vi "Read View VI and FP Refs.vi"(0 "GUI Container in":refnum<class "GUI Container.lvclass">, 5 "View":string, 7 "View Hierarchy Level":i32, 11 "error in (no error)":errorcluster) -> (4 "GUI Container out":refnum<class "GUI Container.lvclass">, 6 "View Status":T1, 8 "VI References":T4, 10 "View Found":bool, 15 "error out":errorcluster)   [LabVIEW 2023, in "GUI Views.lvlib" / "GUI Container.lvclass"]
uses:
  GUI Container.lvclass
  typedefs/VI References.ctl
  typedefs/View Status.ctl
  <vilib>/ActorFramework/Message Enqueuer/Message Enqueuer.lvclass
  typedefs/View Details.ctl
  typedefs/FP Status.ctl
  GUI Container.lvclass/GUI Container.ctl
  <vilib>/ErrorRing/Error Ring.xnode
  <vilib>/Utility/error.llb/Error Cluster From Error Code.vi
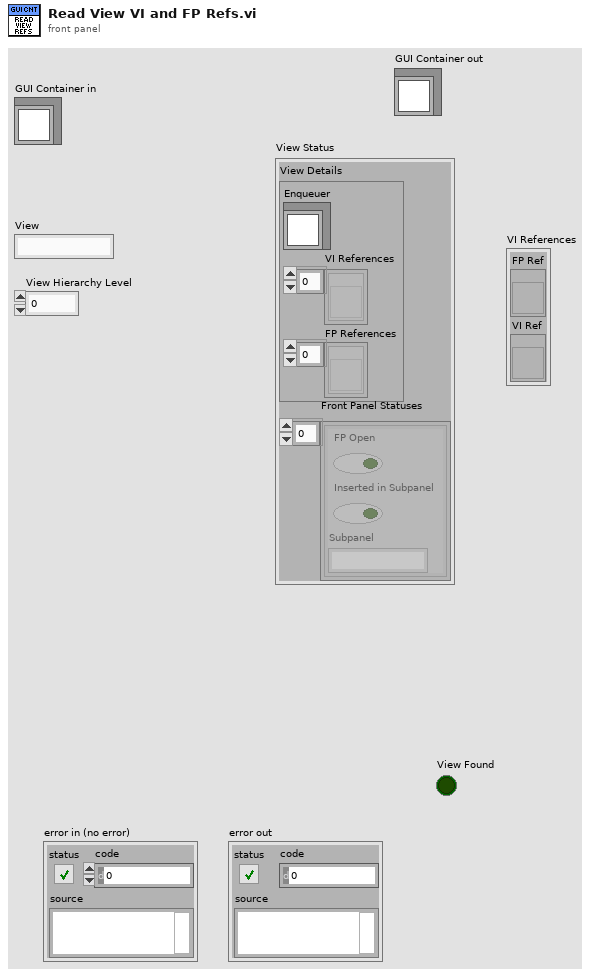
[diagram p1: front panel]
types:
  T1 = typedef "GUI Views.lvlib/GUI Container.lvclass/View Status.ctl" = cluster{"View Details":T2, "Front Panel Statuses":T3[]}
  T2 = typedef "GUI Views.lvlib/GUI Container.lvclass/View Details.ctl" = cluster{"Enqueuer":refnum<class "Message Enqueuer.lvclass">, "VI References":refnum<vi>[], "FP References":refnum<vi>[]}
  T3 = typedef "GUI Views.lvlib/GUI Container.lvclass/FP Status.ctl" = cluster{"FP Open":bool, "Inserted in Subpanel":bool, "Subpanel":string}
  T4 = typedef "GUI Views.lvlib/GUI Container.lvclass/VI References.ctl" = cluster{"FP Ref":refnum<vi>, "VI Ref":refnum<vi>}
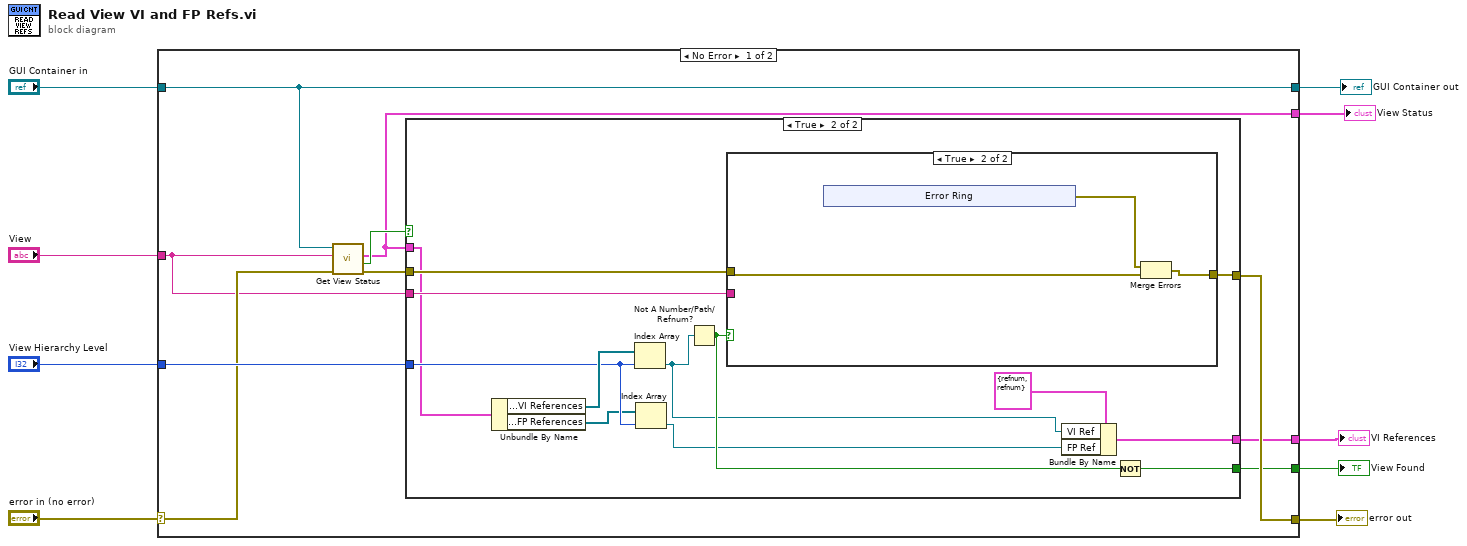
[diagram p0: block diagram]
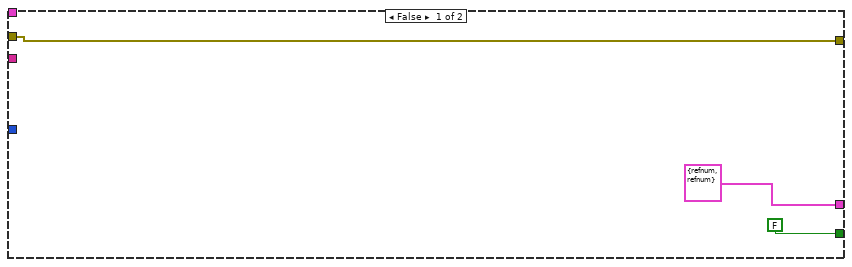
[diagram p2: hidden frame]
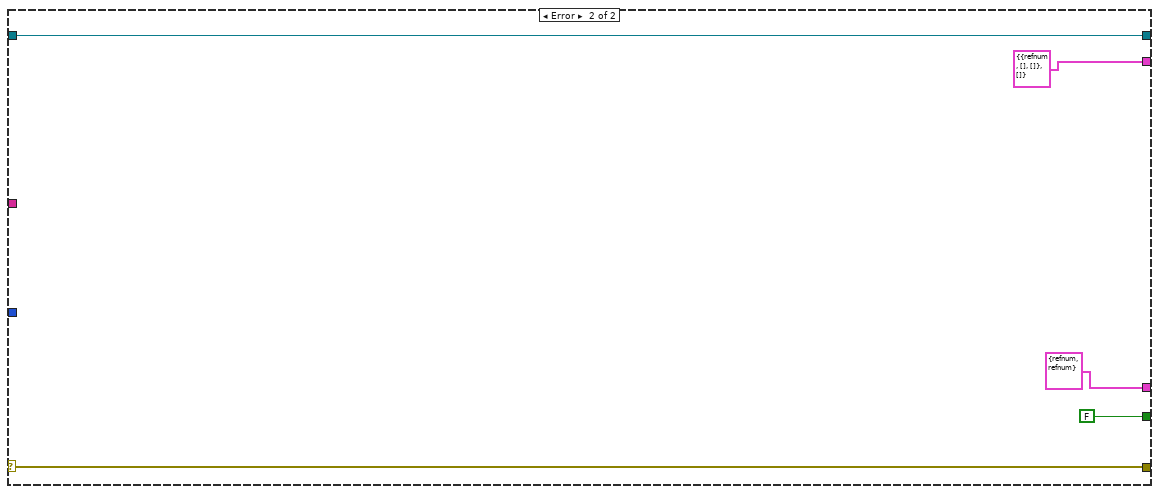
[diagram p4: hidden frame]
diagram:
  n1 = case shown="No Error" "error in (no error)" {
    selector: "error in (no error)" -> [w16 w47]
    tunnel: [w19 w47] -> w9
    tunnel: "GUI Container in" -> [w13 w48]
    tunnel: "View Hierarchy Level" -> [w18 _]
    tunnel: "View" -> [w14 _]
    tunnel: [w13 w48] -> w4
    tunnel: [w17 FALSE] -> w3
    tunnel: [w11 T4 {"FP Ref"=refnum, "VI Ref"=refnum} ("VI References")] -> w2
    tunnel: [w10 T1 {"View Details"={"Enqueuer"=refnum, "VI References"=[], "FP References"=[]}, "Front Panel Statuses"=[]} ("View State")] -> w1
    frame No Error {
      n2 = call "Get View Status.vi"("error in (no error)"=w16, "View"=w14, "GUI Container View in"=w13) -> ("error out"=w15:errorcluster, "View Found"=w12:bool, "View Status"=w10:T1)  [unwired: 5 in, 1 out]
      n3 = case shown="True" w12 {
        tunnel: w15 -> [w22 w34]
        tunnel: w18 -> [_ w32]
        tunnel: [w22 w33] -> w19
        tunnel: w14 -> [_ w31]
        tunnel: [FALSE w23] -> w17
        tunnel: w10 -> [_ w28]
        tunnel: [T4 {"FP Ref"=refnum, "VI Ref"=refnum} ("VI References") w24] -> w11
        frame False {
        }
        frame True {
          n4 = Unbundle By Name(w28) -> ("View Details.VI References"=w35:refnum<vi>[], "View Details.FP References"=w30:refnum<vi>[])
          n5 = Index Array(array=w35, index=w32) -> (element=w25:refnum<vi>)
          n6 = Index Array(array=w30, index=w32) -> (element=w26:refnum<vi>)
          n7 = Not A Number/Path/Refnum?(number/path/refnum=w25) -> (NaN/Path/Refnum?=w29:bool)
          n8 = case shown="True" w29 {
            tunnel: w34 -> [w36 w37]
            tunnel: [w36 w39] -> w33
            tunnel: w31 -> [_ _]
            frame False {
            }
            frame True {
              n9 = xnode "Error Ring"() -> ("error out"=w38:errorcluster)
              n10 = Merge Errors(w38, w37) -> (w39:errorcluster)
            }
          }
          n11 = Bundle By Name(cluster=T4 {"FP Ref"=refnum, "VI Ref"=refnum} ("VI References"), "VI Ref"=w25, "FP Ref"=w26) -> (w24:T4)
          n12 = Not(x=w29) -> (.not. x?=w23:bool)
        }
      }
    }
    frame Error {
    }
  }
  "error out" <- w9
  "GUI Container out" <- w4
  "View Found" <- w3
  "VI References" <- w2
  "View Status" <- w1
